vi "ID.vi"(8 "error in (no error)":errorcluster, 11 "Sensor in":refnum<class "Sensor Config.lvclass">) -> (0 "error out":errorcluster, 2 "ID":string, 3 "Sensor out":refnum<class "Sensor Config.lvclass">)   [LabVIEW 2020, in "VolatusConfig.lvlib" / "Sensor Config.lvclass"]
uses:
  Sensor Config.lvclass
  C:/dev/lv20CE/relink/lv-volatus/VolatusConfig/VolatusConfigElement/VolatusConfigElement.lvclass
  VolatusConfigElement/VolatusConfigElement.lvclass/VolatusConfigElement.ctl
  VolatusConfigElement/Element.vi
  Sensor Config.lvclass/Sensor Config.ctl
  VolatusConfigElement/VolatusConfigElement.lvclass
  lv-cdm/CDM-Config/Config Element/Config Element.lvclass
  C:/dev/lv20CE/relink/lv-volatus/VolatusConfig/Sensor/Sensor Config.lvclass
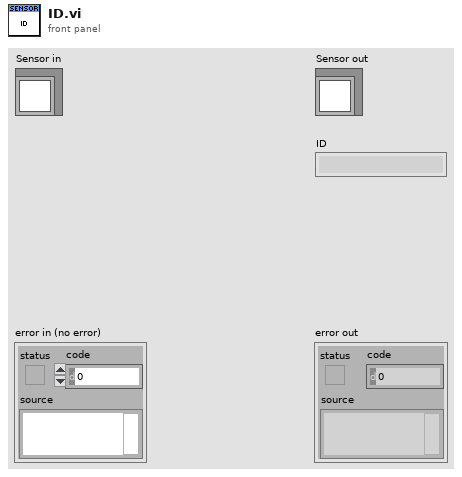
[diagram p1: front panel]
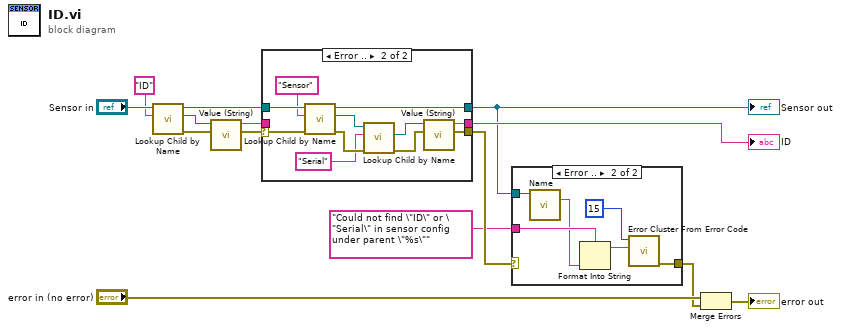
[diagram p0: block diagram]
diagram:
  n1 = call "Lookup Child by Name.vi"("Child Name"="ID", "VolatusConfigElement in"="Sensor in") -> ("error out"=w12:errorcluster, "Child"=w11:refnum<class "Config Element.lvclass">, "VolatusConfigElement out"=w8:refnum<class "Sensor Config.lvclass">)  [unwired: 6 in, 1 out]
  n2 = call "Value (String).vi"("error in (no error)"=w12, "Config Element in"=w11) -> ("error out"=w10:errorcluster, "String Value"=w9:string)  [unwired: 8 in]
  n3 = case shown="Error .." w10 {
    selector: w10 -> [w17 w21]
    tunnel: w9 -> [w16 _]
    tunnel: w8 -> [w15 w28]
    tunnel: [w16 w26] -> w7
    tunnel: [w15 w25] -> w1
    tunnel: [w17 w24] -> w4
    frame No Error {
    }
    frame Error {
      n4 = call "Lookup Child by Name.vi"("error in (no error)"=w21, "Child Name"="Sensor", "VolatusConfigElement in"=w28) -> ("error out"=w22:errorcluster, "Child"=w23:refnum<class "Config Element.lvclass">, "VolatusConfigElement out"=w25:refnum<class "Sensor Config.lvclass">)  [unwired: 5 in, 1 out]
      n5 = call "Lookup Child by Name.vi"("error in (no error)"=w22, "Name"="Serial" ("Child Name"), "Config Element in"=w23) -> ("error out"=w19:errorcluster, "Child"=w20:refnum<class "Config Element.lvclass">)  [unwired: 5 in, 2 out]
      n6 = call "Value (String).vi"("error in (no error)"=w19, "Config Element in"=w20) -> ("error out"=w24:errorcluster, "String Value"=w26:string)  [unwired: 8 in]
    }
  }
  "Sensor out" <- w1
  "ID" <- w7
  n7 = case shown="Error .." w4 {
    selector: w4 -> [w29 _]
    tunnel: "Could not find \"ID\" or \"Serial\" in sensor config under parent \"%s\"" -> [_ w34]
    tunnel: [w29 w32] -> w2
    tunnel: w1 -> [_ w35]
    frame No Error {
    }
    frame Error {
      n8 = call "Name.vi"("VolatusConfigElement in"=w35) -> ("Name"=w33:string)  [unwired: 8 in, 2 out]
      n9 = Format Into String(format string=w34, w33) -> (resulting string=w30:string)  [unwired: 2 in, 1 out]
      n10 = call <vilib>:"Error Cluster From Error Code.vi"("error message (\"\")"=w30, "error code (0)"=15) -> ("error out"=w32:errorcluster)  [unwired: 7 in]
    }
  }
  n11 = Merge Errors("error in (no error)", w2) -> (→"error out":errorcluster)
